vi "Change CO3000 Ant Pol.vi"(8 "error in (no error)":errorcluster caption="에러 입력(에러 없음)", 9 "Mast Index":i32=1, 10 "Antenna Pol":enum16{"H", "V"}(ring), 11 "Instrument Manager 입력":refnum<class "Instrument Manager.lvclass">) -> (0 "error out":errorcluster caption="에러 출력", 3 "Instrument Manager 출력":refnum<class "Instrument Manager.lvclass">)   [LabVIEW 2023, in "Instrument Manager.lvclass"]
uses:
  Instrument Manager.lvclass
  Instrument Manager.lvclass/Instrument Manager.ctl
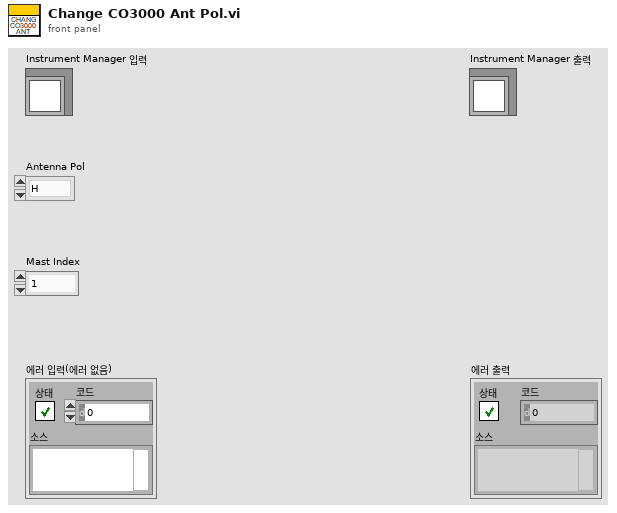
[diagram p1: front panel]
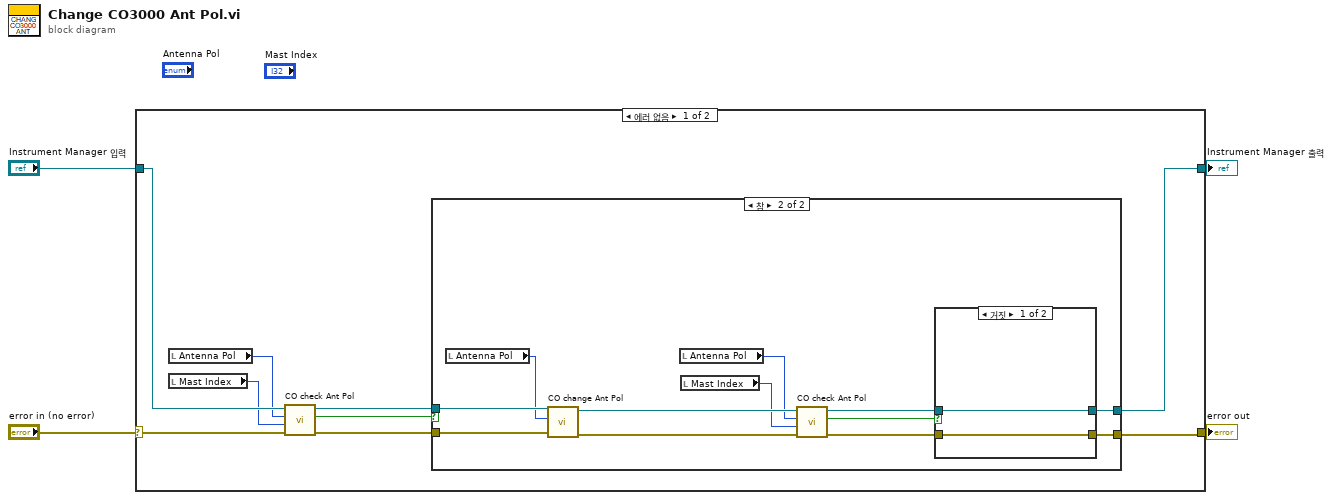
[diagram p0: block diagram]
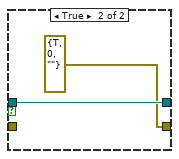
[diagram p3: hidden frame]
diagram:
  n1 = case shown="에러 없음" "error in (no error)" {
    selector: "error in (no error)" -> [w12 w33]
    tunnel: [w8 w33] -> w3
    tunnel: [w7 w32] -> w1
    tunnel: "Instrument Manager 입력" -> [w13 w32]
    frame No Error {
      n2 = local read "Antenna Pol"() -> (w6:enum16{"H", "V"})
      n3 = local read "Mast Index"() -> (w5:i32)
      n4 = call "CO check Ant Pol.vi"("error in (no error)"=w12, "Mast Index"=w5, "Antenna Pol"=w6, "Instrument Manager 입력"=w13) -> ("error out"=w11:errorcluster, "needChange?"=w10:bool, "Instrument Manager 출력"=w9:refnum<class "Instrument Manager.lvclass">)  [unwired: 5 in]
      n5 = case shown="참" w10 {
        tunnel: w11 -> [w15 w26]
        tunnel: w9 -> [w14 w27]
        tunnel: [w15 w20] -> w8
        tunnel: [w14 w19] -> w7
        frame False {
        }
        frame True {
          n6 = local read "Antenna Pol"() -> (w17:enum16{"H", "V"})
          n7 = call "CO change Ant Pol.vi"("error in (no error)"=w26, "Antenna Pol"=w17, "Instrument Manager 입력"=w27) -> ("error out"=w24:errorcluster, "Instrument Manager 출력"=w25:refnum<class "Instrument Manager.lvclass">)  [unwired: 7 in]
          n8 = local read "Antenna Pol"() -> (w18:enum16{"H", "V"})
          n9 = local read "Mast Index"() -> (w16:i32)
          n10 = call "CO check Ant Pol.vi"("error in (no error)"=w24, "Mast Index"=w16, "Antenna Pol"=w18, "Instrument Manager 입력"=w25) -> ("error out"=w21:errorcluster, "needChange?"=w23:bool, "Instrument Manager 출력"=w22:refnum<class "Instrument Manager.lvclass">)  [unwired: 5 in]
          n11 = case shown="거짓" w23 {
            tunnel: w22 -> [w28 w31]
            tunnel: w21 -> [w29 _]
            tunnel: [w29 errorcluster {"status"=TRUE, "code"=0, "source"=""} ("error out")] -> w20
            tunnel: [w28 w31] -> w19
            frame False {
            }
            frame True {
            }
          }
        }
      }
    }
    frame Error {
    }
  }
  "error out" <- w3
  "Instrument Manager 출력" <- w1
